vi "Parse Load SA Manual Param.vi"(8 "error in (no error)":errorcluster caption="에러 입력(에러 없음)", 10 "JSON string":string, 11 "Instrument Manager 입력":refnum<class "Instrument Manager.lvclass">) -> (0 "error out":errorcluster caption="에러 출력", 1 "SA Manual Param":T1={"Start Frequency"=0.0, "Stop Frequency"=0.0, "RBW"=0.0, "VBW"=0.0, "Sweep Point"=0, "Sweep Time"=0.0, "Atten Level"=0.0, "Detector Type"=enum."RMS", "Limit"=0.0}, 2 "Load SA Manual Setting Param":T3, 3 "Instrument Manager 출력":refnum<class "Instrument Manager.lvclass">)   [LabVIEW 2023, in "Instrument Manager.lvclass"]
uses:
  Instrument Manager.lvclass
  Param Definition/Load SA Manual Setting Param.ctl
  Type Definition/SA Manual Param.ctl
  Module/Spectrum Analyzer/TYPE DEFINITION/TYPE Detect Mode Select.ctl
  Instrument Manager.lvclass/Instrument Manager.ctl
  Module/Spectrum Analyzer/Spectrum Analyzer.lvlib
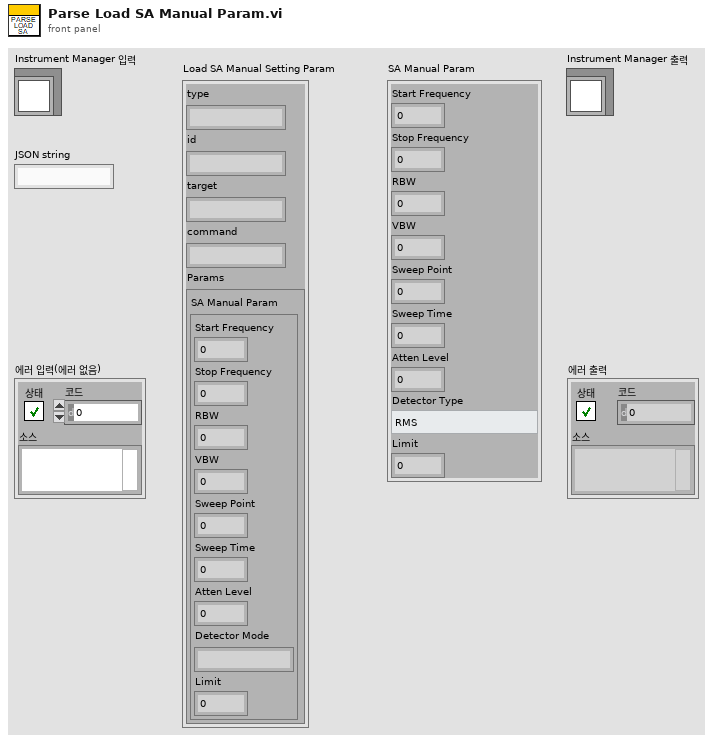
[diagram p1: front panel]
types:
  T1 = typedef "SA Manual Param.ctl" = cluster{"Start Frequency":dbl, "Stop Frequency":dbl, "RBW":dbl, "VBW":dbl, "Sweep Point":u32, "Sweep Time":dbl, "Atten Level":dbl, "Detector Type":T2, "Limit":dbl}
  T2 = typedef "Spectrum Analyzer.lvlib/TYPE Detect Mode Select.ctl" = enum16{"Det Auto (Normal)", "Auto Peak", "Positive Peak", "Negative Peak", "Sample", "RMS", "Average", "Quasipeak", "CISPR Average", "RMS Average"}
  T3 = typedef "Instrument Manager.lvclass/Load SA Manual Setting Param.ctl" = cluster{"type":string, "id":string, "target":string, "command":string, "Params":cluster{"SA Manual Param":cluster{"Start Frequency":dbl, "Stop Frequency":dbl, "RBW":dbl, "VBW":dbl, "Sweep Point":u32, "Sweep Time":dbl, "Atten Level":dbl, "Detector Mode":string, "Limit":dbl}}}
  T4 = cluster{"SA Manual Param":cluster{"Start Frequency":dbl, "Stop Frequency":dbl, "RBW":dbl, "VBW":dbl, "Sweep Point":u32, "Sweep Time":dbl, "Atten Level":dbl, "Detector Mode":string, "Limit":dbl}}
  T5 = cluster{"Start Frequency":dbl, "Stop Frequency":dbl, "RBW":dbl, "VBW":dbl, "Sweep Point":u32, "Sweep Time":dbl, "Atten Level":dbl, "Detector Mode":string, "Limit":dbl}
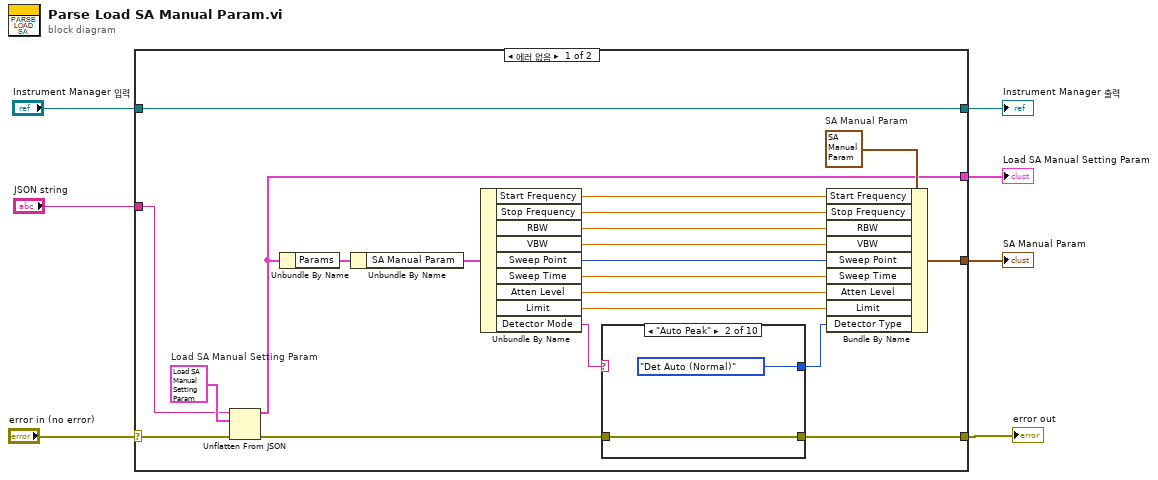
[diagram p0: block diagram]
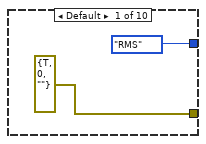
[diagram p2: hidden frame]
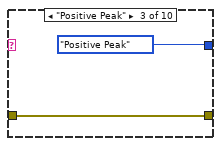
[diagram p3: hidden frame]
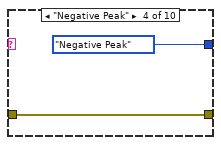
[diagram p4: hidden frame]
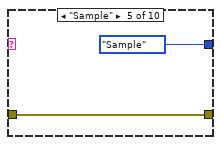
[diagram p5: hidden frame]
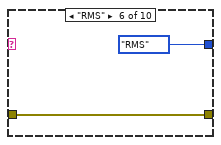
[diagram p6: hidden frame]
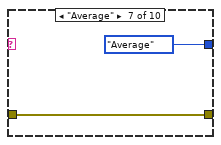
[diagram p7: hidden frame]
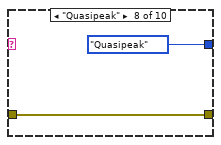
[diagram p8: hidden frame]
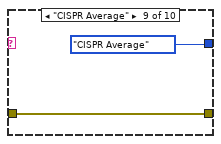
[diagram p9: hidden frame]
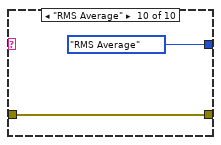
[diagram p10: hidden frame]
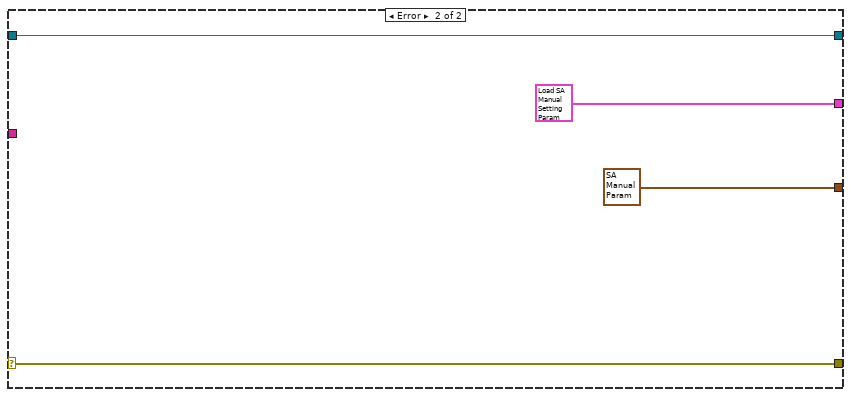
[diagram p11: hidden frame]
diagram:
  n1 = case shown="에러 없음" "error in (no error)" {
    selector: "error in (no error)" -> [w27 w52]
    tunnel: [w8 w52] -> w6
    tunnel: [w28 w51] -> w4
    tunnel: "Instrument Manager 입력" -> [w28 w51]
    tunnel: "JSON string" -> [w25 _]
    tunnel: [w13 T1 {"Start Frequency"=0.0, "Stop Frequency"=0.0, "RBW"=0.0, "VBW"=0.0, "Sweep Point"=0, "Sweep Time"=0.0, "Atten Level"=0.0, "Detector Type"=enum."RMS", "Limit"=0.0} ("SA Manual Param")] -> w2
    tunnel: [w12 T3 {"type"="", "id"="", "target"="", "command"="", "Params"={"SA Manual Param"={"Start Frequency"=0.0, "Stop Frequency"=0.0, "RBW"=0.0, "VBW"=0.0, "Sweep Point"=0, "Sweep Time"=0.0, "Atten Level"=0.0, "Detector Mode"="", "Limit"=0.0}}} ("Load SA Manual Setting Param")] -> w1
    frame No Error {
      w23 = T1 {"Start Frequency"=0.0, "Stop Frequency"=0.0, "RBW"=0.0, "VBW"=0.0, "Sweep Point"=0, "Sweep Time"=0.0, "Atten Level"=0.0, "Detector Type"=enum."RMS", "Limit"=0.0}  # SA Manual Param
      w26 = T3 {"type"="", "id"="", "target"="", "command"="", "Params"={"SA Manual Param"={"Start Frequency"=0.0, "Stop Frequency"=0.0, "RBW"=0.0, "VBW"=0.0, "Sweep Point"=0, "Sweep Time"=0.0, "Atten Level"=0.0, "Detector Mode"="", "Limit"=0.0}}}  # Load SA Manual Setting Param
      n2 = Unflatten From JSON(JSON string=w25, type and defaults=w26, error in (no error)=w27) -> (value=w12:T3, error out=w9:errorcluster)  [unwired: 4 in]
      n3 = Unbundle By Name(w12) -> ("Params"=w24:T4)
      n4 = Unbundle By Name(w24) -> ("SA Manual Param"=w22:T5)
      n5 = Unbundle By Name(w22) -> ("Start Frequency"=w21:dbl, "Stop Frequency"=w20:dbl, "RBW"=w19:dbl, "VBW"=w18:dbl, "Sweep Point"=w17:u32, "Sweep Time"=w16:dbl, "Atten Level"=w15:dbl, "Limit"=w14:dbl, "Detector Mode"=w11:string)
      n6 = case shown="\"Auto Peak\"" w11 {
        tunnel: [TYPE_Detect_Mode_Select."RMS" ("Detector Type") TYPE_Detect_Mode_Select."Det Auto (Normal)" ("Detector Type") TYPE_Detect_Mode_Select."Positive Peak" ("Detector Type") TYPE_Detect_Mode_Select."Negative Peak" ("Detector Type") TYPE_Detect_Mode_Select."Sample" ("Detector Type") TYPE_Detect_Mode_Select."RMS" ("Detector Type") TYPE_Detect_Mode_Select."Average" ("Detector Type") TYPE_Detect_Mode_Select."Quasipeak" ("Detector Type") TYPE_Detect_Mode_Select."CISPR Average" ("Detector Type") TYPE_Detect_Mode_Select."RMS Average" ("Detector Type")] -> w10
        tunnel: w9 -> [_ w31 w33 w35 w37 w39 w41 w43 w45 w47]
        tunnel: [errorcluster {"status"=TRUE, "code"=0, "source"=""} ("error out") w31 w33 w35 w37 w39 w41 w43 w45 w47] -> w8
        frame Default {
        }
        frame "Auto Peak" {
        }
        frame "Positive Peak" {
        }
        frame "Negative Peak" {
        }
        frame "Sample" {
        }
        frame "RMS" {
        }
        frame "Average" {
        }
        frame "Quasipeak" {
        }
        frame "CISPR Average" {
        }
        frame "RMS Average" {
        }
      }
      n7 = Bundle By Name(cluster=w23, "Start Frequency"=w21, "Stop Frequency"=w20, "RBW"=w19, "VBW"=w18, "Sweep Point"=w17, "Sweep Time"=w16, "Atten Level"=w15, "Limit"=w14, "Detector Type"=w10) -> (w13:T1)
    }
    frame Error {
    }
  }
  "error out" <- w6
  "Instrument Manager 출력" <- w4
  "Load SA Manual Setting Param" <- w1
  "SA Manual Param" <- w2
